vi "Ctor.vi"(8 "error in (no error)":errorcluster, 11 "SequenceViewPanel in":refnum<class "SequenceViewPanel.lvclass">) -> (0 "error out":errorcluster, 3 "SequenceViewPanel out":refnum<class "SequenceViewPanel.lvclass">)   [LabVIEW 2020, in "TSnax UI.lvlib" / "SequenceViewPanel.lvclass"]
uses:
  SequenceViewPanel.lvclass
  SequenceViewPanel.lvclass/SequenceViewPanel.ctl
  <vilib>/IlluminatedG/IG OOPanel/OOPanel/Panel/Panel.lvclass
  Ref Data.ctl
  TSnax/SequenceFile/SequenceFile.lvclass
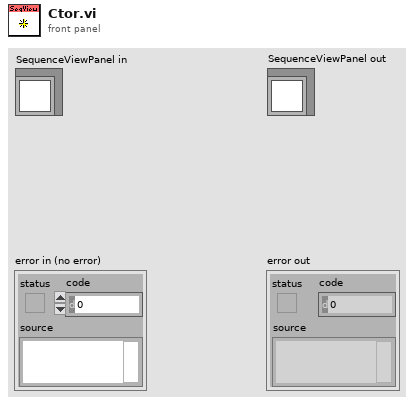
[diagram p1: front panel]
types:
  T1 = typedef "TSnax UI.lvlib/SequenceViewPanel.lvclass/Ref Data.ctl" = cluster{"Insert Line":i32, "SequenceFile":refnum<class "SequenceFile.lvclass">, "Sequence":string, "Trace Marker":i32}
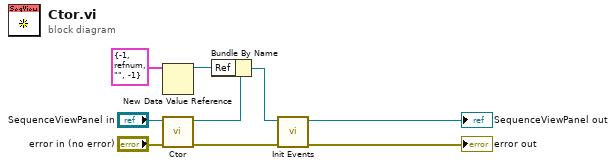
[diagram p0: block diagram]
diagram:
  n1 = New Data Value Reference(data value=T1 {"Insert Line"=-1, "SequenceFile"=refnum, "Sequence"="", "Trace Marker"=-1} ("Ref Data")) -> (data value reference=w3:refnum<data-value>)  [unwired: 1 in, 1 out]
  n2 = call-parent "Ctor.vi"("error in (no error)"="error in (no error)", "Panel in"="SequenceViewPanel in") -> ("error out"=w6:errorcluster, "Panel out"=w8:refnum<class "SequenceViewPanel.lvclass">)  [unwired: 8 in]
  n3 = Bundle By Name(cluster=w8, "Ref"=w3) -> (w4:refnum<class "SequenceViewPanel.lvclass">)
  n4 = call "Init Events.vi"("error in (no error)"=w6, "SequenceViewPanel in"=w4) -> ("error out"=→"error out":errorcluster, "SequenceViewPanel out"=→"SequenceViewPanel out":refnum<class "SequenceViewPanel.lvclass">)  [unwired: 8 in]
